vi "Schedule Guardian Recheck.vi"(8 "error in (no error)":errorcluster, 10 "Guardian ID":string, 11 "Guardian in":refnum<class "Guardian.lvclass">) -> (0 "error out":errorcluster, 3 "Guardian out":refnum<class "Guardian.lvclass">)   [LabVIEW 2020, in "TALOS.lvlib" / "Guardian.lvlib" / "Guardian.lvclass"]
uses:
  Guardian.lvclass
  Guardian Messages/Guardian Died Recheck Msg/Guardian Died Recheck Msg.lvclass
  builds/Actor Framework PPL/Actor Framework.lvlibp/1abvi3w/vi.lib/ActorFramework/Actor/Actor.lvclass
  builds/Actor Framework PPL/Actor Framework.lvlibp
  builds/Actor Framework PPL/Actor Framework.lvlibp/1abvi3w/vi.lib/ActorFramework/Message Enqueuer/Message Priority.ctl
  builds/Actor Framework PPL/Actor Framework.lvlibp/1abvi3w/vi.lib/ActorFramework/Message Enqueuer/Message Enqueuer.lvclass
  TALOS.lvlib
  C:/LabVIEW Code/TALOS/talos/Ancestor/Ancestor/Ancestor.lvclass
  C:/LabVIEW Code/TALOS/builds/Actor Framework PPL/Actor Framework.lvlibp/1abvi3w/vi.lib/ActorFramework/Actor/Actor.lvclass
  C:/LabVIEW Code/TALOS/talos/Guardian/Guardian/Guardian.lvclass
  C:/LabVIEW Code/TALOS/builds/Actor Framework PPL/Actor Framework.lvlibp/1abvi3w/vi.lib/ActorFramework/Message/Message.lvclass
  C:/LabVIEW Code/TALOS/talos/Guardian/Guardian Messages/Guardian Died Recheck Msg/Guardian Died Recheck Msg.lvclass
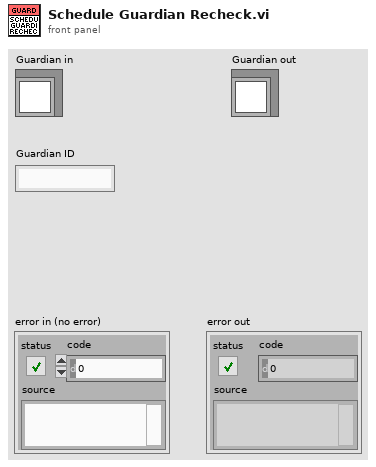
[diagram p1: front panel]
types:
  T1 = typedef "Actor Framework.lvlibp/Message Enqueuer.lvclass/Message Priority.ctl" = enum16{"Low", "Normal", "High"}
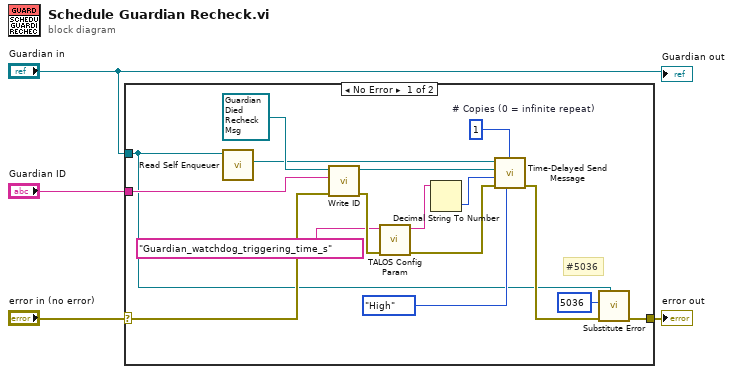
[diagram p0: block diagram]
diagram:
  n1 = case shown="No Error" "error in (no error)" {
    selector: "error in (no error)" -> [w18 w21]
    tunnel: "Guardian in" -> [w6 _]
    tunnel: [w7 w21] -> w4
    tunnel: "Guardian ID" -> [w19 _]
    frame No Error {
      w15 = u32 1  # # Copies (0 = infinite repeat)
      # "#5036"
      n2 = call "Read Self Enqueuer.vi"("Actor"=w6) -> ("Self Enqueuer"=w16:refnum<class "Message Enqueuer.lvclass">)  [unwired: 10 in]
      n3 = call "Write ID.vi"("error in (no error)"=w18, "ID"=w19, "Guardian Died Recheck Msg in"=refnum<class "Guardian Died Recheck Msg.lvclass"> refnum ("Guardian.lvlib:Guardian Died Recheck Msg.lvclass")) -> ("error out"=w12:errorcluster, "Guardian Died Recheck Msg out"=w17:refnum<class "Guardian Died Recheck Msg.lvclass">)  [unwired: 7 in]
      n4 = call "TALOS Config Param.vi"("error in (no error)"=w12, "Parameter Name"="Guardian_watchdog_triggering_time_s") -> ("error out"=w11:errorcluster, "Output"=w10:string)  [unwired: 8 in]
      n5 = Decimal String To Number(string=w10) -> (number=w13:i32)  [unwired: 2 in, 1 out]
      n6 = call "Time-Delayed Send Message.vi"("Message Priority (Normal)"=Message_Priority."High", "# Copies (0 = infinite repeat)"=w15, "error in (no error)"=w11, "Milliseconds To Wait"=w13, "Message"=w17, "Message Enqueuer"=w16) -> ("error out"=w8:errorcluster)  [unwired: 4 in, 1 out]
      n7 = call "Substitute Error.vi"("LabVIEW Object"=w6, "error in (no error)"=w8, "Error Code"=5036) -> ("error out"=w7:errorcluster)  [unwired: 8 in]
    }
    frame Error {
    }
  }
  "error out" <- w4
  "Guardian out" <- "Guardian in"
